vi "configuration UI.vi"() -> ()   [LabVIEW 2013, in "control module editor.lvclass"]
doc: "All child modules share this same UI. The UI allows for the configuration of Channels, Parameters, and Error Handling."
uses:
  control module editor.lvclass
  <vilib>/NI/Configuration Framework/Node/NodeRef.ctl
  <vilib>/NI/Configuration Framework/Node/NISE_CEF_Node.lvclass
  <vilib>/NI/AMC/Message Queue.ctl
  <vilib>/NI/AMC/Message.ctl
  <vilib>/NI/Tools/Keyed Array/KeyedArray.ctl
  <vilib>/NI/Configuration Framework/Node/UserEventRef.ctl
  <vilib>/NI/Configuration Framework/Controls/EventCluster.ctl
  configuration/error classification setting.ctl
  <vilib>/NI/Tag Bus Module Framework/runtime/error classification.ctl
  <vilib>/NI/Configuration Framework/Node/RefreshUIEvent.ctl
  <vilib>/NI/Configuration Framework/Node/CacheState.ctl
  <vilib>/NI/Configuration Framework/Node/StopEvent.ctl
  <vilib>/NI/Configuration Framework/Node/NodeChangeEvent.ctl
  Table API/Available Tag Menu/channel action event.ctl
  Table API/Available Tag Menu/dialog output action.ctl
  <vilib>/NI/Tag Bus Module Framework/channel/TBM channel.lvclass
  <vilib>/NI/Tag Bus/tag/tag descriptor.lvclass
  Table API/Table Manager/Call Back Ref Type Def.ctl
  Configuration Editor/Classes/Engine Parent/Engine Parent Editor Node.lvclass
  Configuration Editor/Classes/Module editor node/module editor node.lvclass
  Table API/Table Manager/references.ctl
  Table API/Table Manager/Menu Definition.ctl
  Table API/Table Manager/Menu Options.ctl
  configuration/control module configuration.lvclass
  Table API/Listbox/Multi Column Listbox.lvclass
  configuration/control module configuration.lvclass/control module configuration.ctl
  <vilib>/NI/Tag Bus Module Framework/module configuration/TBM module configuration.lvclass
  <vilib>/NI/Configuration Framework/serializable configuration/NISE_CEF_serializable configuration.lvclass/NISE_CEF_serializable configuration.ctl
  <vilib>/NI/Tag Bus Module Framework/channel/channel classification.ctl
  configuration/Write error classifications.vi
  Configuration Editor/Classes/Module editor node/Read Module Configuration.vi
  read fixed channel configuration.vi
  <vilib>/Utility/LVClass/Get LV Class Name.vi
  <vilib>/NI/Configuration Framework/error generator/NISE_error generator.vi
  <vilib>/NI/Configuration Framework/serializable configuration/NISE_CEF_serializable configuration.lvclass
  <vilib>/NI/Configuration Framework/NISE_CEF_TreeControl.lvlib
  Table API/Table Manager.lvlib
  <vilib>/NI/DCAF UI Toolkit/Controls/DCAF UI Elements.lvlib
  <vilib>/NI/Tools/Keyed Array/Tools_KeyedArray.lvlib
  <vilib>/NI/AMC/AMC.lvlib
  Table API/Table Manager/Table Manager.lvclass
  <vilib>/NI/Tag Bus Module Framework/runtime/TBM module execution interface.lvclass
panel:
  in  "Enum":i32
  in  "user event out":refnum<user-event>
  in  "Top Level Tab Control":T1(tab)
  in  "Channels Listbox":i32(listbox)
  in  "mapall":bool
  in  "mapwriters":bool
  in  "Parameters Listbox":i32(listbox)
  in  "error classifications":T2[](array[typedef])
  in  "node change":T4
  in  "stop event":T5
  in  "cache state":T6
  in  "refresh UI":T7
  in  "user event":T8
  in  "main queue":T9
  in  "node ref":T10
  # "(Single-Click to Edit)"
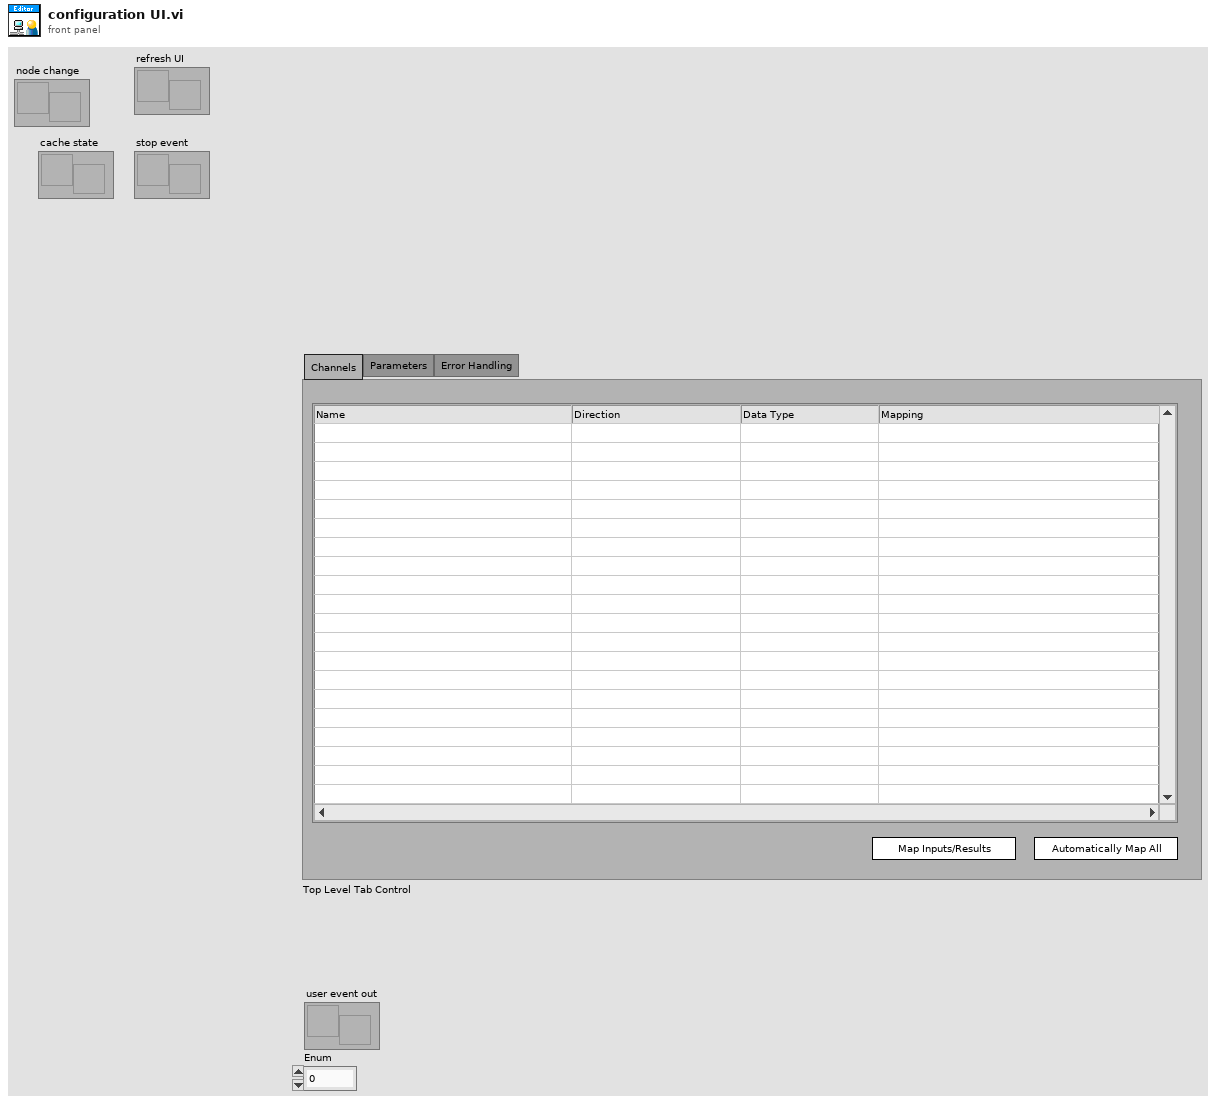
[diagram p1: front panel]
types:
  T1 = enum32{"Channels", "Parameters", "Error Handling"}
  T2 = typedef "control module configuration.lvclass/error classification setting.ctl" = cluster{"code":i32, "error classification":T3}
  T3 = typedef "TBM module execution interface.lvclass/error classification.ctl" = enum16{"unknown", "none", "trivial", "recoverable", "critical"}
  T4 = typedef "NISE_CEF_Node.lvclass/NodeChangeEvent.ctl" = refnum<user-event>
  T5 = typedef "NISE_CEF_Node.lvclass/StopEvent.ctl" = refnum<user-event>
  T6 = typedef "NISE_CEF_Node.lvclass/CacheState.ctl" = refnum<user-event>
  T7 = typedef "NISE_CEF_Node.lvclass/RefreshUIEvent.ctl" = refnum<user-event>
  T8 = typedef "NISE_CEF_Node.lvclass/UserEventRef.ctl" = refnum<user-event>
  T9 = typedef "AMC.lvlib/Message Queue.ctl" = refnum<queue>
  T10 = typedef "NISE_CEF_Node.lvclass/NodeRef.ctl" = refnum<data-value>
  T11 = typedef "Table Manager.lvlib/Table Manager.lvclass/Menu Definition.ctl" = cluster{"Menu Name":string, "Menu Options":T12}
  T12 = typedef "Table Manager.lvlib/Table Manager.lvclass/Menu Options.ctl" = enum16{"Always Show", "Show When Used", "Show When Empty"}
  T13 = typedef "Table Manager.lvlib/Table Manager.lvclass/references.ctl" = cluster{"stop event":T5, "refresh UI":T7, "cache state":T6, "node change":T4, "user event out":refnum<user-event>, "main queue":T9, "user event":T8}
  T14 = typedef "Table Manager.lvlib/Column.lvclass/Column Descriptor.ctl" = cluster{"name":string, "caption":string, "Column Type":T15, "Params":string, "AutoSizeMode":i32, "FillWeight":sgl, "MinWidth":u32, "tooltip":string, "Enum Reference":refnum<vi>, "Channel suffix":string, "Read Only":bool, "Call Back VI":T16, "DT Dependency":i32, "name dependency":i32, "data type":T17, "Custom Column":refnum<class "Column.lvclass">}
  T15 = typedef "Table Manager.lvlib/Column.lvclass/Column Type.ctl" = enum16{"String", "Mapping", "Enum", "Custom"}
  T16 = typedef "Table Manager.lvlib/Table Manager.lvclass/Call Back Ref Type Def.ctl" = refnum<vi>
  T17 = typedef "tag bus.lvlib/tag descriptor.lvclass/Data Type.ctl" = enum16{"Double", "Single", "I64", "I32", "I16", "I8", "U64", "U32", "U16", "U8", "Boolean", "String", "Array of Double", "Array of Single", "Array of I64", "Array of I32", "Array of I16", "Array of I8", "Array of U64", "Array of U32", "Array of U16", "Array of U8", "Array of Boolean", "Array of String"}
  T18 = typedef "Table Manager.lvlib/Table Manager.lvclass/object ref.ctl" = cluster{"engine":refnum<data-value>, "Node Ref":refnum<data-value>}
  T19 = typedef "Table Manager.lvlib/Table Manager.lvclass/Table Events.ctl" = cluster{"Menu Selection":refnum<user-event>}
  T20 = typedef "NISE_CEF_TreeControl.lvlib/EventCluster.ctl" = cluster{"command":string, "data":string}
  T21 = typedef "TBM channel.lvclass/channel classification.ctl" = enum16{"input data", "output data", "processing parameter", "processing result"}
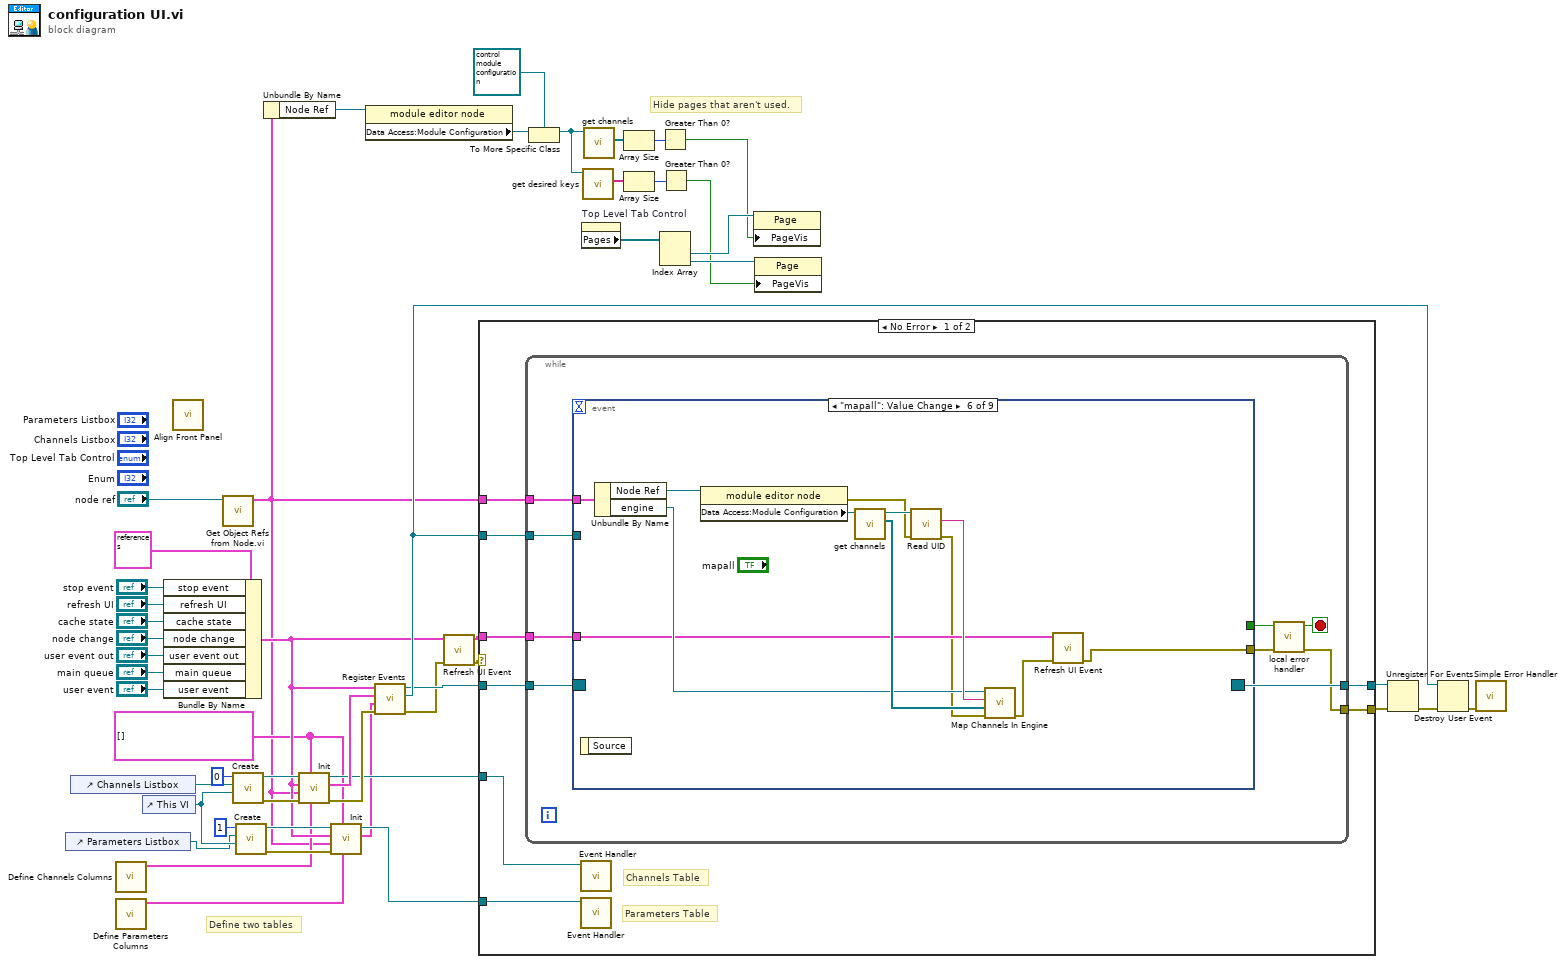
[diagram p0: block diagram]
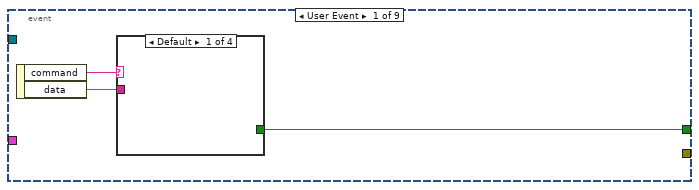
[diagram p2: hidden frame]
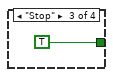
[diagram p4: hidden frame]
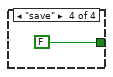
[diagram p5: hidden frame]
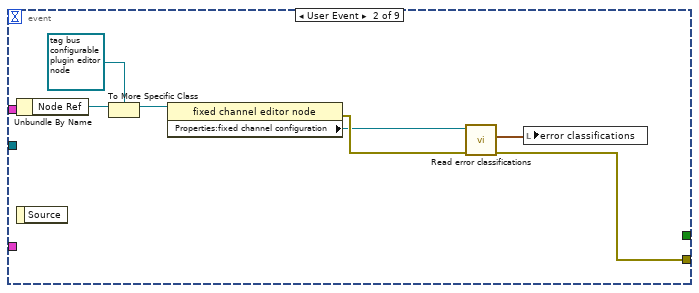
[diagram p6: hidden frame]
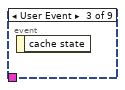
[diagram p7: hidden frame]
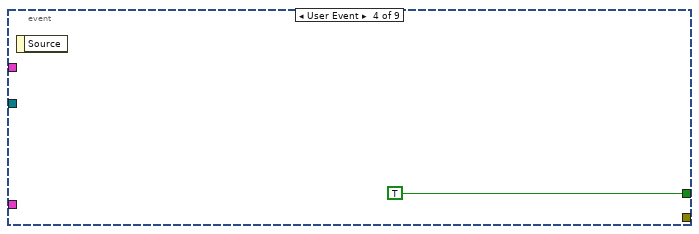
[diagram p8: hidden frame]
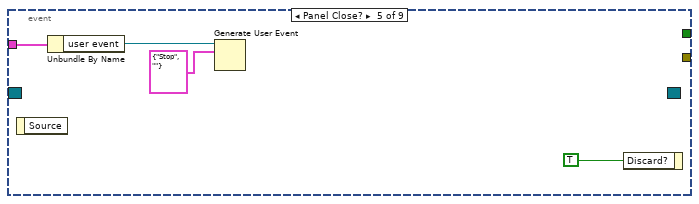
[diagram p9: hidden frame]
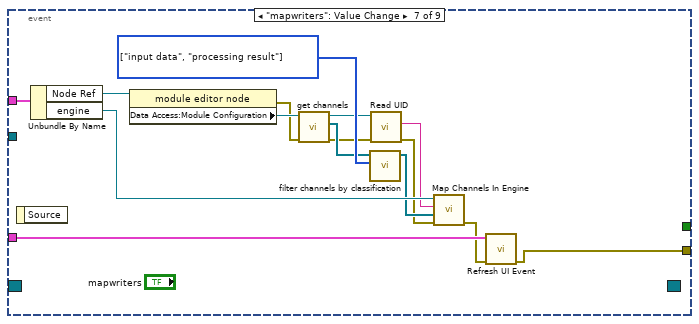
[diagram p10: hidden frame]
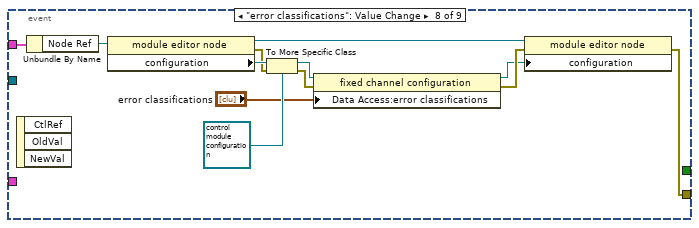
[diagram p11: hidden frame]
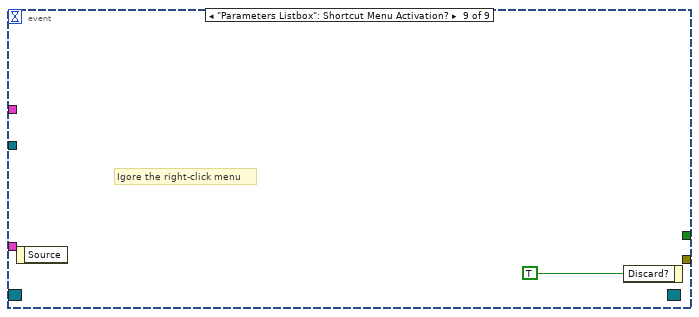
[diagram p12: hidden frame]
diagram:
  w15 = T11[] [] ("Right-Click Menu")
  # "Define two tables"
  # "Hide pages that aren't used."
  n1 = control-ref of="Parameters Listbox"() -> (w18:refnum<vi>)
  n2 = control-ref of="Channels Listbox"() -> (w26:refnum<vi>)
  n3 = call "Define Channels Columns.vi"() -> ("Column Descriptors"=w17:T14[])  [unwired: 11 in]
  n4 = call "Define Parameters Columns.vi"() -> ("Column Descriptors"=w16:T14[])  [unwired: 11 in]
  n5 = control-ref of="This VI"() -> (w22:refnum<vi>)
  n6 = Bundle By Name(cluster=T13 {"stop event"=refnum, "refresh UI"=refnum, "cache state"=refnum, "node change"=refnum, "user event out"=refnum, "main queue"=refnum, "user event"=refnum} ("Event References"), "stop event"="stop event", "refresh UI"="refresh UI", "cache state"="cache state", "node change"="node change", "user event out"="user event out", "main queue"="main queue", "user event"="user event") -> (w19:T13)
  n7 = call <vilib>:"Align Front Panel.vi"() -> ()  [unwired: 10 in, 2 out]
  n8 = call "Get Object Refs from Node.vi.vi"("node ref"="node ref") -> ("Node object refs"=w7:T18)  [unwired: 9 in, 1 out]
  n9 = call "Create.vi"("Top VI"=w22, "Listbox"=w26, "Index"=0) -> ("error out"=w29:errorcluster, "reference out"=w30:refnum<class "Multi Column Listbox.lvclass">)  [unwired: 7 in]
  n10 = call "Create.vi"("Top VI"=w22, "Listbox"=w18, "Index"=1) -> ("error out"=w25:errorcluster, "reference out"=w24:refnum<class "Multi Column Listbox.lvclass">)  [unwired: 7 in]
  n11 = Unbundle By Name(w7) -> ("Node Ref"=w5:refnum<data-value>)
  n12 = call-dynamic "Init.vi"("Column Descriptors"=w17, "Right-Click Menu"=w15, "error in (no error)"=w29, "Node object refs"=w7, "Event References"=w19, "Multi Column Listbox in"=w30) -> ("error out"=w28:errorcluster, "Table Events"=w40:T19, "Multi Column Listbox out"=w27:refnum<class "Multi Column Listbox.lvclass">)  [unwired: 3 in]
  n13 = call-dynamic "Init.vi"("Column Descriptors"=w16, "Right-Click Menu"=w15, "error in (no error)"=w25, "Node object refs"=w7, "Event References"=w19, "Multi Column Listbox in"=w24) -> ("Table Events"=w20:T19, "Multi Column Listbox out"=w21:refnum<class "Multi Column Listbox.lvclass">)  [unwired: 3 in, 1 out]
  n14 = property class="module editor node"(reference=w5) -> ("Data Access:Module Configuration"=w6:refnum<class "TBM module configuration.lvclass">)  [unwired: 1 in, 2 out]
  n15 = call "Register Events.vi"("error in (no error)"=w28, "Parameters Table Events"=w20, "Channels Table Events"=w40, "Event References"=w19) -> ("error out"=w33:errorcluster, "Channel Action"=w39:refnum<user-event>, "Event Registration Refnum"=w38:refnum<event-registration>)  [unwired: 5 in]
  n16 = call "Refresh UI Event.vi"("error in (no error)"=w33, "Event References"=w19) -> ("error out"=w34:errorcluster, "Event References out"=w32:T13)  [unwired: 8 in]
  n17 = case shown="No Error" w34 {
    selector: w34 -> [_ w126]
    tunnel: w38 -> [w58 w125]
    tunnel: [w57 w125] -> w50
    tunnel: [w55 w126] -> w49
    tunnel: w39 -> [w56 _]
    tunnel: w7 -> [w54 _]
    tunnel: w32 -> [w53 _]
    tunnel: w27 -> [w52 _]
    tunnel: w21 -> [w51 _]
    frame No Error {
      # "Parameters Table"
      # "Channels Table"
      n18 = while {
        tunnel: w58 -> [w67]
        tunnel: [w66] -> w57
        tunnel: w56 -> [w65]
        tunnel: [w61] -> w55
        tunnel: w54 -> [w60]
        tunnel: w53 -> [w59]
        stop <- w63 stop-if-true
        n19 = event shown="[5] \"mapall\": Value Change" {
          selector: w67 -> [_ _ _ _ _ _ _ _ _]
          dyn-events: [_ _ _ _ _ _ _ _ _] -> w66
          timeout: _ -> [_ _ _ _ _ _ _ _ _]
          tunnel: [w70 _ _ TRUE _ _ _ _ _] -> w64
          tunnel: [_ w77 _ _ _ w91 w107 w123 _] -> w62
          tunnel: w65 -> [_ _ _ _ _ _ _ _ _]
          tunnel: w60 -> [_ w80 _ _ _ w95 w108 w122 _]
          tunnel: w59 -> [_ _ _ _ w83 w90 w106 _ _]
          event User Event {
            n20 = event-data() -> ("command"=w69:string, "data"=w68:string)  [unwired: 1 in]
            n21 = case shown="Default" w69 {
              tunnel: [_ _ TRUE FALSE] -> w70
              tunnel: w68 -> [_ _ _ _]
              frame Default {
              }
              frame "Refresh" {
              }
              frame "Stop" {
              }
              frame "save" {
              }
            }
          }
          event User Event {
            n22 = Unbundle By Name(w80) -> ("Node Ref"=w78:refnum<data-value>)
            n23 = event-data() -> ()  [unwired: 1 in, 1 out]
            n24 = To More Specific Class(target class=refnum<data-value> refnum ("data value reference"), reference=w78) -> (specific class reference=w76:refnum<data-value>)  [unwired: 1 in, 1 out]
            n25 = property class="fixed channel editor node"(reference=w76) -> (error out=w75:errorcluster, "Properties:fixed channel configuration"=w73:refnum<class "control module configuration.lvclass">)  [unwired: 1 in, 1 out]
            n26 = call "Read error classifications.vi"("error in"=w75, "control module configuration in"=w73) -> ("error out"=w77:errorcluster, "error classifications"=w74:T2[])  [unwired: 7 in, 1 out]
            n27 = local write "error classifications"(w74) -> ()
          }
          event User Event {
            n28 = event-data() -> ()  [unwired: 1 in, 1 out]
          }
          event User Event {
            n29 = event-data() -> ()  [unwired: 1 in, 1 out]
          }
          event Panel Close? {
            n30 = event-data() -> ()  [unwired: 1 in, 1 out]
            n31 = Unbundle By Name(w83) -> ("user event"=w82:T8)
            n32 = Generate User Event(user event=w82, event data cluster=T20 {"command"="Stop", "data"=""} ("event data")) -> ()  [unwired: 2 in, 2 out]
            n33 = event-data("Discard?"=TRUE) -> ()  [unwired: 1 in, 1 out]
          }
          event "mapall": Value Change {
            n34 = event-data() -> ()  [unwired: 1 in, 1 out]
            n35 = Unbundle By Name(w95) -> ("Node Ref"=w94:refnum<data-value>, "engine"=w93:refnum<data-value>)
            n36 = property class="module editor node"(reference=w94) -> (error out=w87:errorcluster, "Data Access:Module Configuration"=w89:refnum<class "TBM module configuration.lvclass">)  [unwired: 1 in, 1 out]
            n37 = call-dynamic "get channels.vi"("module configuration in"=w89) -> ("channels"=w97:refnum<class "TBM channel.lvclass">[], "module configuration out"=w88:refnum<class "TBM module configuration.lvclass">)  [unwired: 9 in]
            n38 = call <vilib>:"Read UID.vi"("error in"=w87, "configuration in"=w88) -> ("error out"=w86:errorcluster, "instance id"=w96:string)  [unwired: 7 in, 1 out]
            n39 = call "Map Channels In Engine.vi"("error in (no error)"=w86, "channels"=w97, "instance id"=w96, "Engine DVR"=w93) -> ("error out"=w92:errorcluster)  [unwired: 7 in]
            n40 = call "Refresh UI Event.vi"("error in (no error)"=w92, "Event References"=w90) -> ("error out"=w91:errorcluster)  [unwired: 8 in, 1 out]
          }
          event "mapwriters": Value Change {
            w111 = T21[] [enum."input data", enum."processing result"] items=["input data", "output data", "processing parameter", "processing result"] ("allowed classifications")
            n41 = event-data() -> ()  [unwired: 1 in, 1 out]
            n42 = Unbundle By Name(w108) -> ("Node Ref"=w109:refnum<data-value>, "engine"=w105:refnum<data-value>)
            n43 = property class="module editor node"(reference=w109) -> (error out=w98:errorcluster, "Data Access:Module Configuration"=w100:refnum<class "TBM module configuration.lvclass">)  [unwired: 1 in, 1 out]
            n44 = call-dynamic "get channels.vi"("module configuration in"=w100) -> ("channels"=w110:refnum<class "TBM channel.lvclass">[], "module configuration out"=w99:refnum<class "TBM module configuration.lvclass">)  [unwired: 9 in]
            n45 = call <vilib>:"filter channels by classification.vi"("allowed classifications"=w111, "channels in"=w110) -> ("channels out"=w103:refnum<class "TBM channel.lvclass">[])  [unwired: 9 in]
            n46 = call <vilib>:"Read UID.vi"("error in"=w98, "configuration in"=w99) -> ("error out"=w102:errorcluster, "instance id"=w104:string)  [unwired: 7 in, 1 out]
            n47 = call "Map Channels In Engine.vi"("error in (no error)"=w102, "channels"=w103, "instance id"=w104, "Engine DVR"=w105) -> ("error out"=w101:errorcluster)  [unwired: 7 in]
            n48 = call "Refresh UI Event.vi"("error in (no error)"=w101, "Event References"=w106) -> ("error out"=w107:errorcluster)  [unwired: 8 in, 1 out]
          }
          event "error classifications": Value Change {
            n49 = event-data() -> ()  [unwired: 1 in, 3 out]
            n50 = Unbundle By Name(w122) -> ("Node Ref"=w117:refnum<data-value>)
            n51 = property class="module editor node"(reference=w117) -> (reference out=w121:refnum<data-value>, error out=w113:errorcluster, "configuration"=w116:refnum<class "NISE_CEF_serializable configuration.lvclass">)  [unwired: 1 in]
            n52 = To More Specific Class(target class=refnum<class "control module configuration.lvclass"> refnum ("fixed channel configuration"), reference=w116, error in=w113) -> (specific class reference=w118:refnum<class "control module configuration.lvclass">, error out=w112:errorcluster)
            n53 = property class="fixed channel configuration"(reference=w118, error in=w112, "Data Access:error classifications"="error classifications") -> (reference out=w119:refnum<class "control module configuration.lvclass">, error out=w120:errorcluster)
            n54 = property class="module editor node"(reference=w121, error in=w120, "configuration"=w119) -> (error out=w123:errorcluster)  [unwired: 1 out]
          }
          event "Parameters Listbox": Shortcut Menu Activation? {
            # "Igore the right-click menu"
            n55 = event-data() -> ()  [unwired: 1 in, 1 out]
            n56 = event-data("Discard?"=TRUE) -> ()  [unwired: 1 in, 1 out]
          }
        }
        n57 = call "local error handler.vi"("error in (no error)"=w62, "Stop in"=w64) -> ("error out"=w61:errorcluster, "Stop out"=w63:bool)  [unwired: 8 in]
      }
      n58 = call-dynamic "Event Handler.vi"("Listbox in"=w52) -> ()  [unwired: 9 in, 2 out]
      n59 = call-dynamic "Event Handler.vi"("Listbox in"=w51) -> ()  [unwired: 9 in, 2 out]
    }
    frame Error {
    }
  }
  n60 = To More Specific Class(target class=refnum<class "control module configuration.lvclass"> refnum ("fixed channel configuration"), reference=w6) -> (specific class reference=w3:refnum<class "control module configuration.lvclass">)  [unwired: 1 in, 1 out]
  n61 = property on="Top Level Tab Control" class="TabCtl (strict)"() -> ("Pages"=w8:refnum<vi>[])  [unwired: 2 in, 2 out]
  n62 = call-dynamic "get desired keys.vi"("fixed channel configuration in"=w3) -> ("desired keys"=w11:string[])  [unwired: 8 in, 2 out]
  n63 = call-dynamic "get channels.vi"("fixed channel configuration in"=w3) -> ("channels"=w14:refnum<class "TBM channel.lvclass">[])  [unwired: 9 in, 1 out]
  n64 = Array Size(array=w14) -> (size(s)=w13:i32)
  n65 = Array Size(array=w11) -> (size(s)=w12:i32)
  n66 = Greater Than 0?(x=w13) -> (x > 0?=w2:bool)
  n67 = Index Array(array=w8) -> (element #1=w9:refnum<vi>, element #2=w10:refnum<vi>)  [unwired: 2 in]
  n68 = Greater Than 0?(x=w12) -> (x > 0?=w1:bool)
  n69 = property class="Page"(reference=w9, "PageVis"=w2) -> ()  [unwired: 1 in, 2 out]
  n70 = property class="Page"(reference=w10, "PageVis"=w1) -> ()  [unwired: 1 in, 2 out]
  n71 = Unregister For Events(event registration refnum=w50, error in=w49) -> (error out=w48:errorcluster)
  n72 = Destroy User Event(user event=w39, error in=w48) -> (error out=w47:errorcluster)
  n73 = call <vilib>:"Simple Error Handler.vi"("error in (no error)"=w47) -> ()  [unwired: 4 in, 5 out]
